vi "Build Parameters.vi"(10 "Parameters":T2[](array[typedef])) -> (2 "Scenarios":T1(array[cluster]))   [LabVIEW 2026, in "Generate VI Names.lvclass"]
doc: "This helper function simplifies the syntax of creating parameters."
uses:
  Generate VI Names.lvclass
  Parameters.ctl
  <vilib>/Astemes/LUnit Parameterized/Parameterized Test Case/Parameterized Test Case.lvclass
  Generate VI Names.lvclass/Generate VI Names.ctl
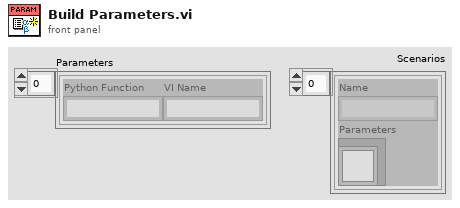
[diagram p1: front panel]
types:
  T1 = cluster{"Name":string, "Parameters":refnum<class "Parameterized Test Case.lvclass">}[]
  T2 = typedef "Generate VI Names.lvclass/Parameters.ctl" = cluster{"Python Function":string, "VI Name":string}
  T3 = cluster{"Scenario":string, "Parameters":refnum<class "Generate VI Names.lvclass">}
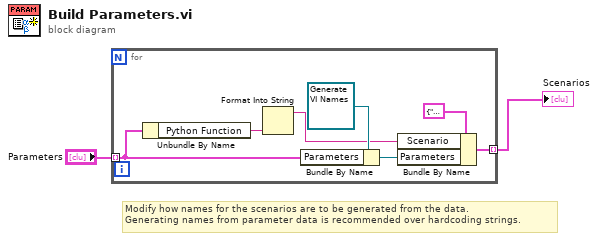
[diagram p0: block diagram]
diagram:
  # "Modify how names for the scenarios are to be generated from the data.\nGenerating names from parameter data is recommended over hardcoding strings."
  n1 = for {
    tunnel: [w7] -> w1 mode=indexing
    tunnel: "Parameters" -> [w5] mode=indexing
    n2 = Unbundle By Name(w5) -> ("Python Function"=w4:string)
    n3 = Format Into String(w4) -> (resulting string=w3:string)  [unwired: 3 in, 1 out]
    n4 = Bundle By Name(cluster=refnum<class "Generate VI Names.lvclass"> refnum ("Parameters"), "Parameters"=w5) -> (w8:refnum<class "Generate VI Names.lvclass">)
    n5 = Bundle By Name(cluster=T3 {"Scenario"="", "Parameters"=refnum}, "Scenario"=w3, "Parameters"=w8) -> (w7:T3)
  }
  "Scenarios" <- w1
